vi "Own20261012_SetFormulaExpression.vi"() -> ()   [LabVIEW 2024]
panel:
  out "error out":errorcluster caption="错误输出"
  in  "expression":string
  in  "formula_id":u32
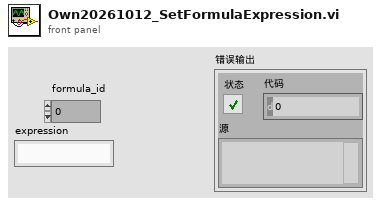
[diagram p1: front panel]
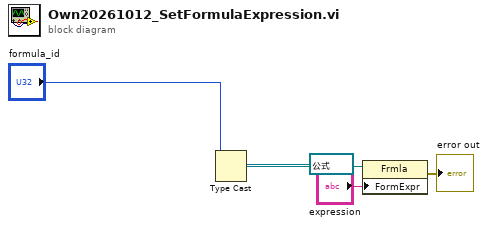
[diagram p0: block diagram]
diagram:
  n1 = Type Cast(type=refnum<vi> refnum ("引用"), x="formula_id") -> (*(type *) &x=w3:refnum<vi>)
  n2 = property class="Frmla"(reference=w3, "FormExpr"="expression") -> (error out=→"error out":errorcluster)  [unwired: 1 in, 1 out]
